vi "ECAT Generate OD For FPGA IOV.vi"(8 "error in":errorcluster, 10 "Product Code":u32, 11 "Input bitfile path":path) -> (0 "error out":errorcluster, 1 "OD object structure":T1[](array[typedef]) {"od_index" format="%.0x"; "lptr_name" format="%.0x"; "lptr_data" format="%.0x"; "lptr_entry" format="%.0x"; "DataInfo"."u8Array" format="%.0x"}, 3 "File Byte Array":u8[](array[numeric]), 5 "IOVs from bitfile":T2(array[cluster]) {"address" format="%.0x"})   [LabVIEW 2020, in "SEECD System Explorer.lvlib"]
uses:
  SEECD System Explorer.lvlib
  <vilib>/LabVIEW Targets/FPGA/ECat/subVIs/FPGAParsingVIs/niECATODInfoStructure.ctl
panel:
  # "This VI wraps FPGA bitfile into FoE file and generate FPGA IOV OD information from bitfile.\nThen this VI merge wipeback FoE block,  FPGA bitstream FoE block and FPGA IOV OD FoE block into one FoE file."
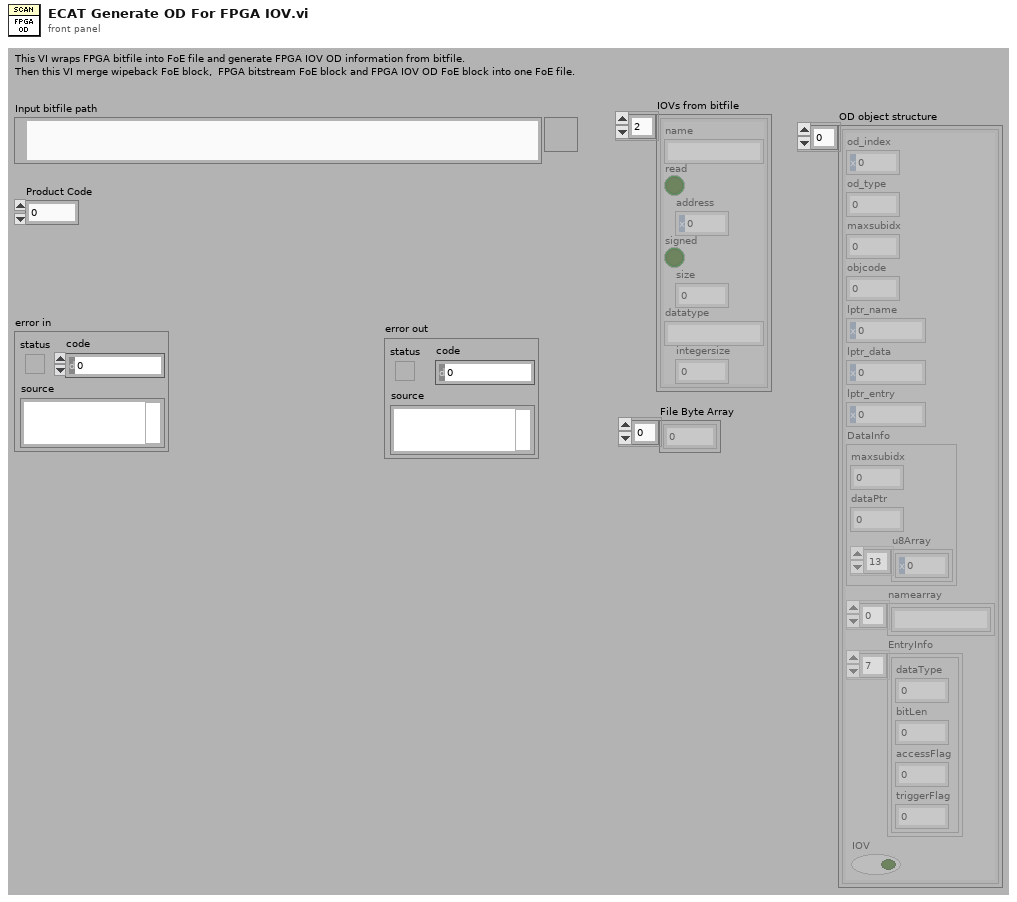
[diagram p1: front panel]
types:
  T1 = typedef "niECATODInfoStructure.ctl" = cluster{"od_index":u32, "od_type":u16, "maxsubidx":u8, "objcode":u8, "lptr_name":u32, "lptr_data":u32, "lptr_entry":u32, "DataInfo":cluster{"maxsubidx":u32, "dataPtr":u32, "u8Array":u8[]}, "namearray":string[], "EntryInfo":cluster{"dataType":u16, "bitLen":u16, "accessFlag":u16, "triggerFlag":u16}[], "IOV":bool}
  T2 = cluster{"name":string, "read":bool, "address":u32, "signed":bool, "size":u32, "datatype":string, "integersize":i32}[]
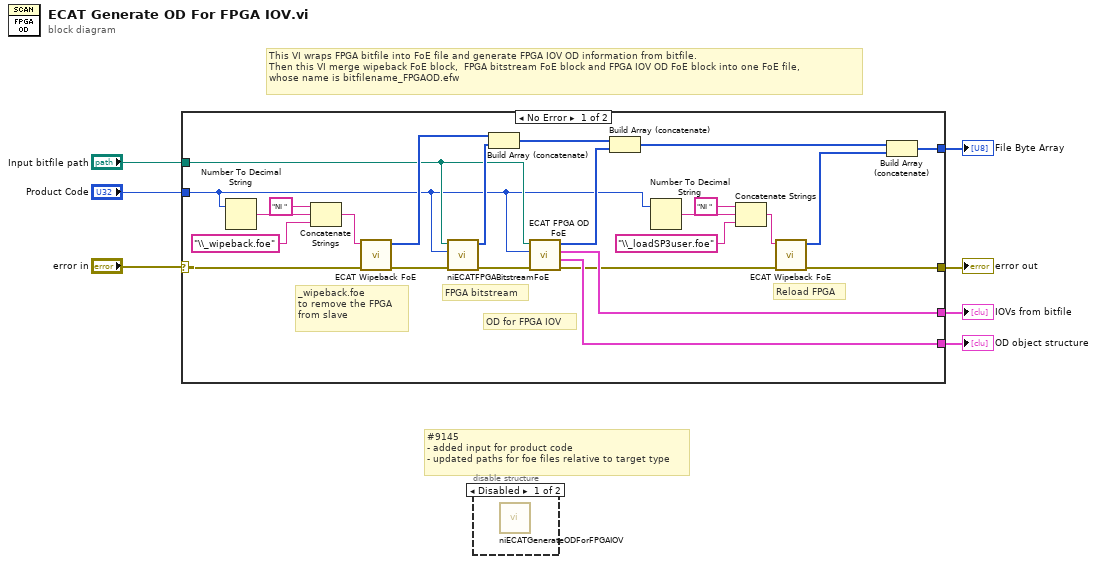
[diagram p0: block diagram]
diagram:
  # "#9145\n- added input for product code\n- updated paths for foe files relative to target type"
  # "This VI wraps FPGA bitfile into FoE file and generate FPGA IOV OD information from bitfile.\nThen this VI merge wipeback FoE block,  FPGA bitstream FoE block and FPGA IOV OD FoE block into one FoE file,\nwhose name is bitfilename_FPGAOD.efw"
  n1 = case shown="No Error" "error in" {
    selector: "error in" -> [w12 w32]
    tunnel: [w8 w32] -> w7
    tunnel: "Input bitfile path" -> [w19 _]
    tunnel: [w18 _] -> w4
    tunnel: [w29 _] -> w3
    tunnel: [w24 _] -> w2
    tunnel: "Product Code" -> [w15 _]
    frame No Error {
      # "Reload FPGA"
      # "FPGA bitstream"
      # "OD for FPGA IOV"
      # "_wipeback.foe\nto remove the FPGA \nfrom slave"
      n2 = Number To Decimal String(number=w15) -> (decimal integer string=w22:string)  [unwired: 1 in]
      n3 = Concatenate Strings("NI " ("string"), w22, "\\_wipeback.foe" ("name or relative path")) -> (w20:string)
      n4 = call "ECAT Wipeback FoE.vi"("error in"=w12, "FoE Command"=w20) -> ("error out"=w11:errorcluster, "Output byte array"=w28:u8[])  [unwired: 8 in]
      n5 = call <vilib>:"niECATFPGABitstreamFoE.vi"("error in"=w11, "Product Code"=w15, "Input bitfile path"=w19) -> ("error out"=w10:errorcluster, "Output Byte array"=w25:u8[])  [unwired: 7 in]
      n6 = Build Array (concatenate)(w28, w25) -> (w27:u8[])
      n7 = call "ECAT FPGA OD FoE.vi"("error in"=w10, "Product Code"=w15, "Input bitfile path"=w19) -> ("error out"=w9:errorcluster, "OD object structure"=w18:T1[], "IOVs from bitfile"=w29:T2, "Output Byte array"=w30:u8[])  [unwired: 5 in]
      n8 = Build Array (concatenate)(w27, w30) -> (w31:u8[])
      n9 = Number To Decimal String(number=w15) -> (decimal integer string=w17:string)  [unwired: 1 in]
      n10 = Concatenate Strings("NI " ("string"), w17, "\\_loadSP3user.foe" ("name or relative path")) -> (w13:string)
      n11 = call "ECAT Wipeback FoE.vi"("error in"=w9, "FoE Command"=w13) -> ("error out"=w8:errorcluster, "Output byte array"=w26:u8[])  [unwired: 8 in]
      n12 = Build Array (concatenate)(w31, w26) -> (w24:u8[])
    }
    frame Error {
    }
  }
  "error out" <- w7
  "IOVs from bitfile" <- w3
  "OD object structure" <- w4
  "File Byte Array" <- w2
  n13 = disable-structure shown="Disabled" {
    frame Disabled {
      n14 = call <vilib>:"niECATGenerateODForFPGAIOV.vi"() -> ()  [unwired: 7 in, 5 out]
    }
    frame Enabled {
    }
  }
